vi "Measurement UI.vi"() -> ()   [LabVIEW 2025, in "Automotive Ethernet Frame Generator UI.lvlib"]
uses:
  Automotive Ethernet Frame Generator UI.lvlib
  Automotive Ethernet Frame Generator/OOB gRPC Client/OOB gRPC Client.lvlib
  <vilib>/gRPC/LabVIEW gRPC Library/Shared/grpcId.ctl
  <vilib>/gRPC/LabVIEW gRPC Library/grpc-lvsupport-release.lvlib
panel:
  out "OOB gRPC Port":i32
  out "STATUS":string
  in  "CYCLE?":bool
  in  "PAUSE PCAP PLAYBACK":bool
  in  "PCAP PLAYBACK":bool
  in  "PATH":path
  out "Protocol Layer 2":T1
  out "Payload":string
  in  "SEND FRAME":bool
  out "INTERFACE NAME":refnum<k21>
  out "SENT PACKETS":i32
  out "TC10 POWER MODE":bool
  in  "SEND TC10 COMMAND":bool
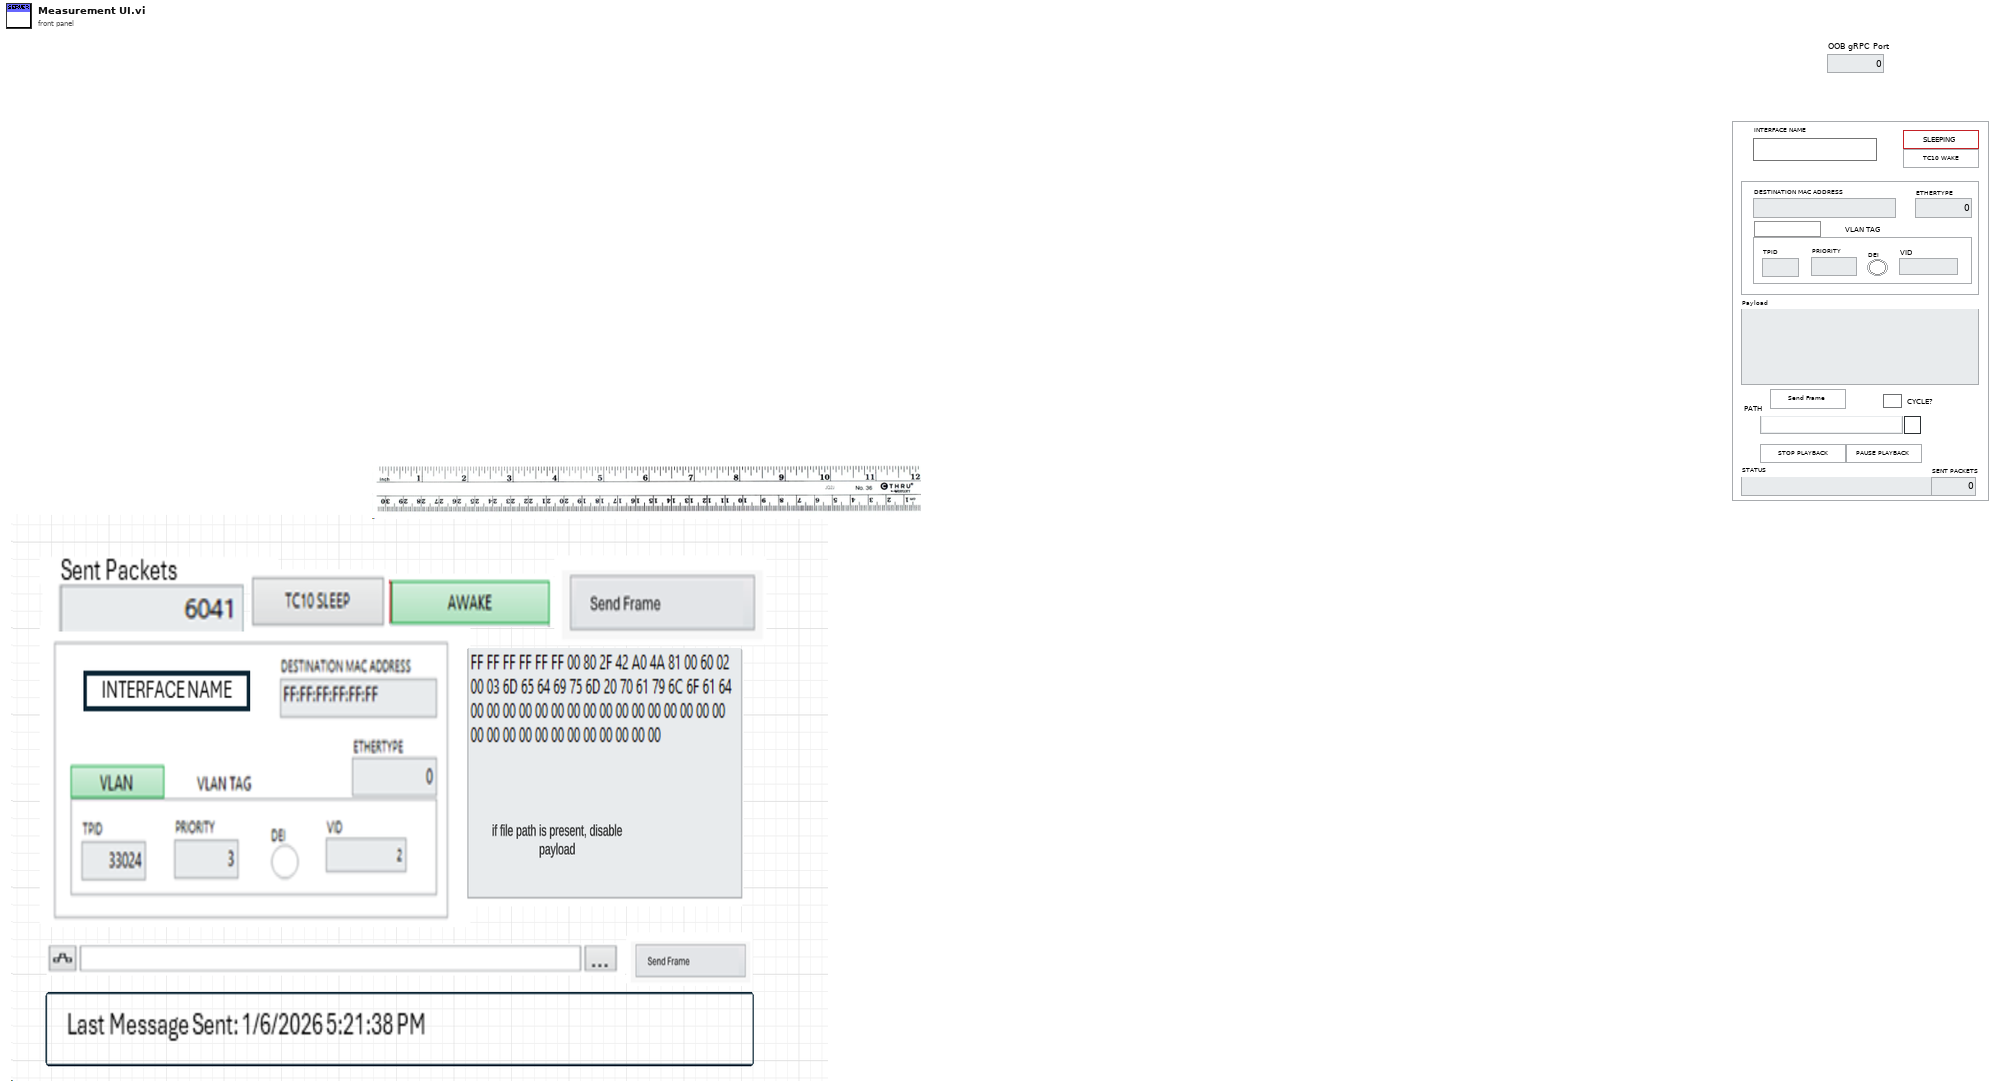
[diagram p1: front panel]
types:
  T1 = cluster{"Has VLAN":bool, "VLAN TAG":cluster{"TPID":u16, "PRIORITY":u8, "DEI":bool, "VID":u16}, "DESTINATION MAC ADDRESS":string, "ETHERTYPE":u16}
  T2 = typedef "grpc-lvsupport-release.lvlib/grpcId.ctl" = u64
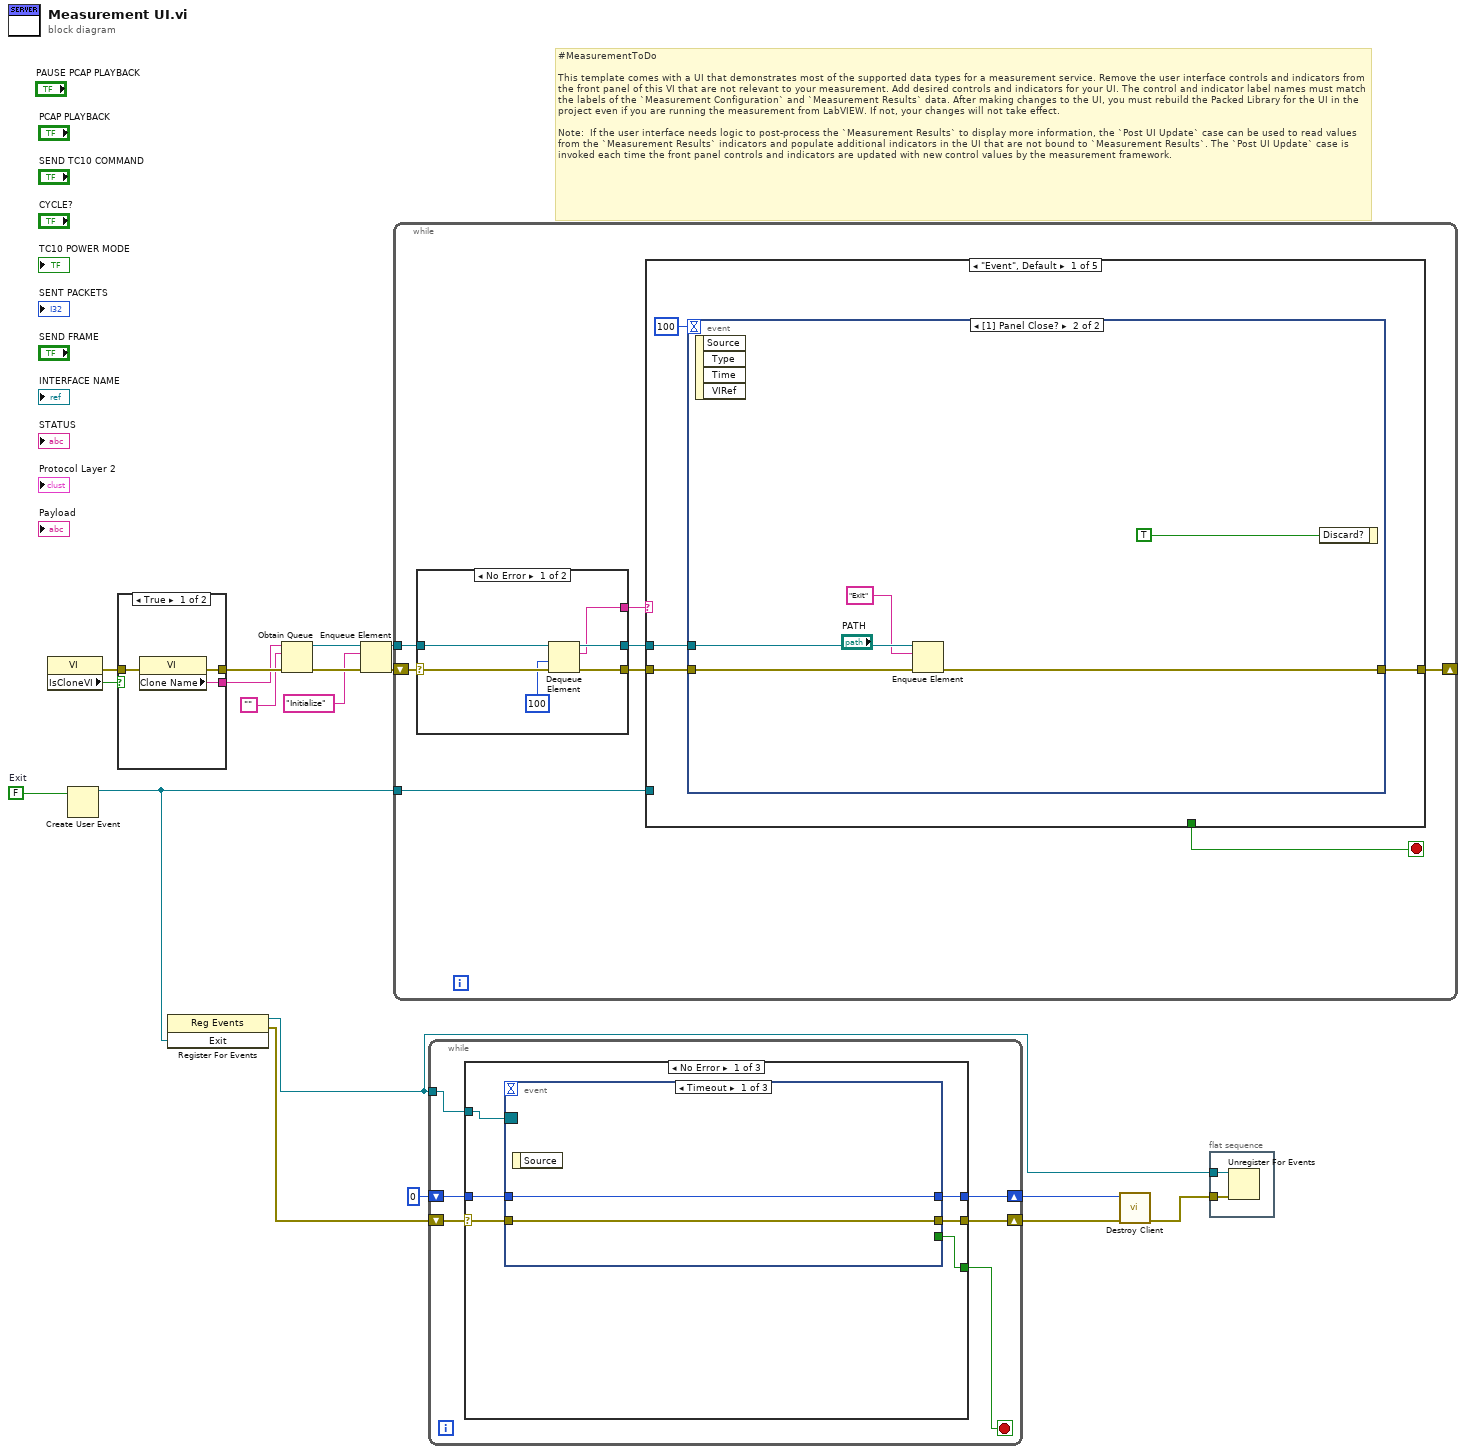
[diagram p0: block diagram]
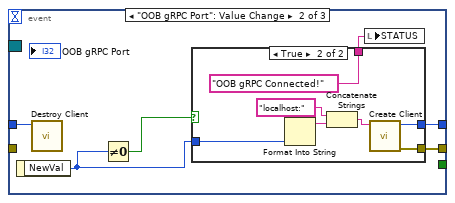
[diagram p2: hidden frame]
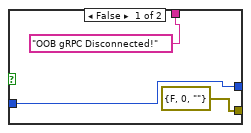
[diagram p3: hidden frame]
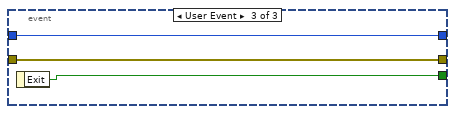
[diagram p4: hidden frame]
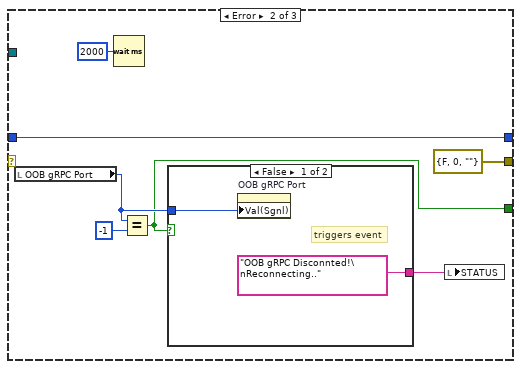
[diagram p5: hidden frame]
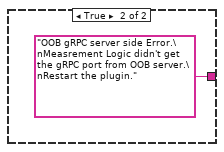
[diagram p6: hidden frame]
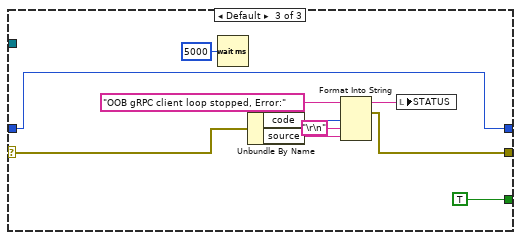
[diagram p7: hidden frame]
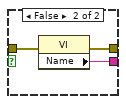
[diagram p8: hidden frame]
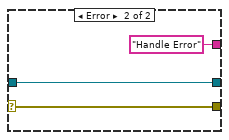
[diagram p9: hidden frame]
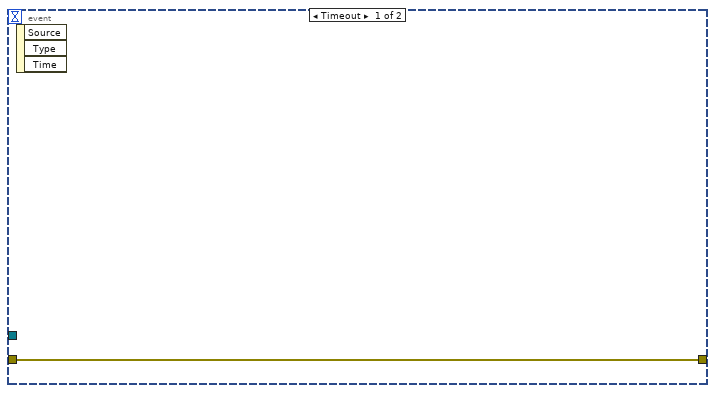
[diagram p10: hidden frame]
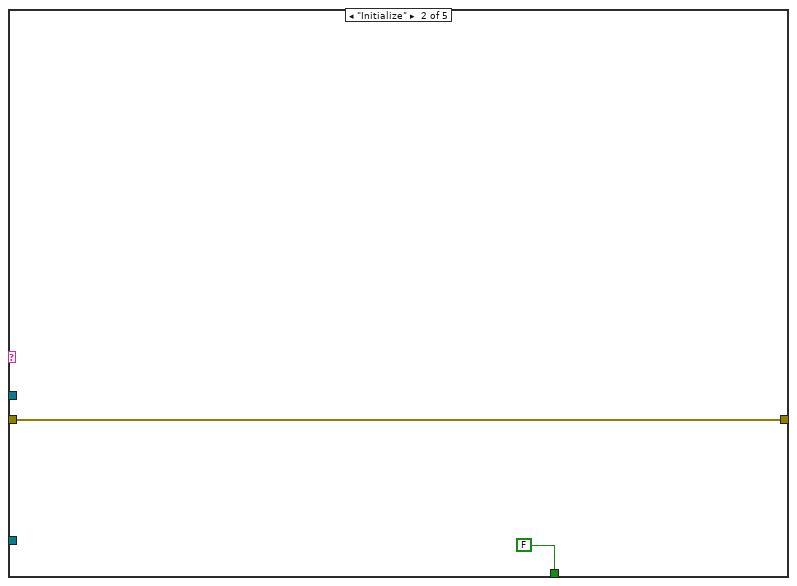
[diagram p11: hidden frame]
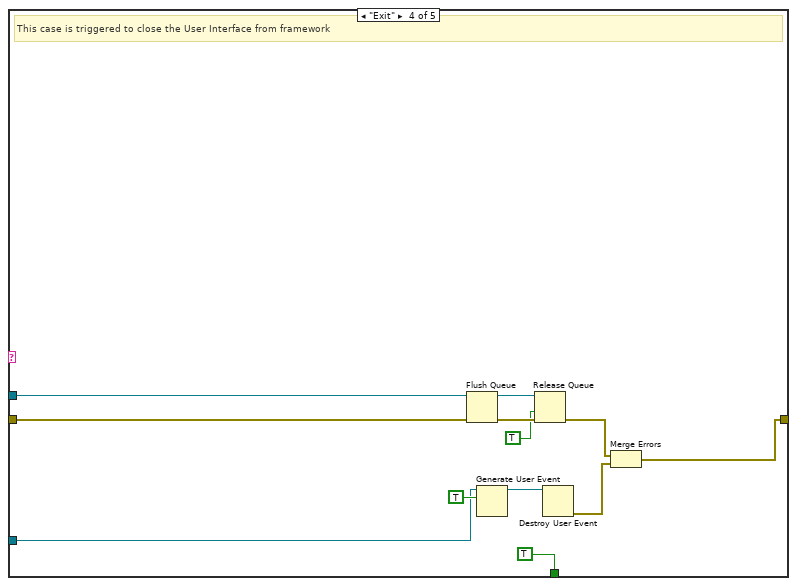
[diagram p13: hidden frame]
diagram:
  w1 = FALSE  # Exit
  # "#MeasurementToDo  \n\nThis template comes with a UI that demonstrates most of the supported data types for a measurement service. Remove the user interface controls and indicators from the front panel of this VI that are not relevant to your measurement. Add desired controls and indicators for your UI. The control and indicator label names must match the labels of the `Measurement Configuration` and `Measurement Results` data. After making changes to the UI, you must rebuild the Packed Library for the UI in the project even if you are running the measurement from LabVIEW. If not, your changes will not take effect.\n\nNote:  If the user interface needs logic to post-process the `Measurement Results` to display more information, the `Post UI Update` case can be used to read values from the `Measurement Results` indicators and populate additional indicators in the UI that are not bound to `Measurement Results`. The `Post UI Update` case is invoked each time the front panel controls and indicators are updated with new control values by the measurement framework."
  n1 = property class="VI"() -> (error out=w9:errorcluster, "IsCloneVI"=w10:bool)  [unwired: 2 in, 1 out]
  n2 = Create User Event(user event datatype=w1) -> (user event=w8:refnum<user-event>)  [unwired: 1 in, 1 out]
  n3 = case shown="True" w10 {
    tunnel: [w21 w24] -> w18
    tunnel: [w20 w23] -> w17
    tunnel: w9 -> [w19 w22]
    frame True {
      n4 = property class="VI"(error in=w19) -> (error out=w21:errorcluster, "Clone Name"=w20:string)  [unwired: 1 in, 1 out]
    }
    frame False {
      n5 = property class="VI"(error in=w22) -> (error out=w24:errorcluster, "Name"=w23:string)  [unwired: 1 in, 1 out]
    }
  }
  n6 = register-events(w8) -> (reference out=w5:refnum<event-registration>, error out=w7:errorcluster)  [unwired: 2 in]
  n7 = Obtain Queue(name (unnamed)=w17, element data type="", error in (no error)=w18) -> (queue out=w14:refnum<queue>, error out=w16:errorcluster)  [unwired: 2 in, 1 out]
  n8 = Enqueue Element(queue=w14, element="Initialize", error in (no error)=w16) -> (queue out=w13:refnum<queue>, error out=w15:errorcluster)  [unwired: 1 in, 1 out]
  n9 = while {
    shift-right: [w27] -> _
    shift-left: w15 -> [w32]
    tunnel: w13 -> [w30]
    tunnel: w8 -> [w25]
    stop <- w26 stop-if-true
    n10 = case shown="No Error" w32 {
      selector: w32 -> [w38 w41]
      tunnel: [w37 w41] -> w31
      tunnel: w30 -> [w36 w40]
      tunnel: [w35 w40] -> w29
      tunnel: [w34 "Handle Error"] -> w28
      frame No Error {
        n11 = Dequeue Element(queue=w36, timeout in ms (-1)=100, error in (no error)=w38) -> (queue out=w35:refnum<queue>, element=w34:string, error out=w37:errorcluster)  [unwired: 1 out]
      }
      frame Error {
      }
    }
    n12 = case shown="\"Event\", Default" w28 {
      tunnel: w31 -> [w44 w53 w54 w66 w67]
      tunnel: w29 -> [w42 _ _ w64 _]
      tunnel: [w45 w53 w54 w55 w67] -> w27
      tunnel: [_ FALSE _ TRUE _] -> w26
      tunnel: w25 -> [_ _ _ w56 _]
      frame "Event", Default {
        n13 = event shown="[1] Panel Close?" {
          selector: _ -> [_ _]
          dyn-events: _ -> [_ _]
          timeout: 100 -> [_ _]
          tunnel: [w46 w49] -> w45
          tunnel: w44 -> [w46 w50]
          tunnel: w42 -> [_ w48]
          event Timeout {
            n14 = event-data() -> ()  [unwired: 1 in, 3 out]
          }
          event Panel Close? {
            n15 = event-data() -> ()  [unwired: 1 in, 4 out]
            n16 = Enqueue Element(queue=w48, element="Exit", error in (no error)=w50) -> (error out=w49:errorcluster)  [unwired: 1 in, 2 out]
            n17 = event-data("Discard?"=TRUE) -> ()  [unwired: 1 in, 1 out]
          }
        }
      }
      frame "Initialize" {
      }
      frame "Post UI Update" {
        # "This case will be triggered, after framework updates the User interface with result values."
      }
      frame "Exit" {
        # "This case is triggered to close the User Interface from framework"
        n18 = Flush Queue(queue=w64, error in (no error)=w66) -> (queue out=w63:refnum<queue>, error out=w62:errorcluster)  [unwired: 1 out]
        n19 = Generate User Event(user event=w56, event data cluster=TRUE ("event data")) -> (user event out=w59:refnum<user-event>)  [unwired: 2 in, 1 out]
        n20 = Release Queue(queue=w63, force destroy? (F)=TRUE, error in (no error)=w62) -> (error out=w58:errorcluster)  [unwired: 2 out]
        n21 = Destroy User Event(user event=w59) -> (error out=w57:errorcluster)  [unwired: 1 in]
        n22 = Merge Errors(w58, w57) -> (w55:errorcluster)
      }
      frame "Handle Error" {
      }
    }
  }
  n23 = while {
    tunnel: w5 -> [w68]
    shift-right: [w72] -> w4
    shift-left: w7 -> [w73]
    shift-right: [w71] -> w3
    shift-left: T2 0 ("gRPC ID Out") -> [w70]
    stop <- w69 stop-if-true
    n24 = case shown="No Error" w73 {
      selector: w73 -> [w76 _ w114]
      tunnel: [w79 errorcluster {"status"=FALSE, "code"=0, "source"=""} ("error IO") w113] -> w72
      tunnel: [w78 w107 w115] -> w71
      tunnel: w70 -> [w77 w107 w115]
      tunnel: [w75 w101 TRUE] -> w69
      tunnel: w68 -> [w74 _ _]
      frame No Error {
        n25 = event shown="[0] Timeout" {
          selector: w74 -> [_ _ _]
          dyn-events: _ -> [_ _ _]
          timeout: _ -> [_ _ _]
          tunnel: [w80 w85 w99] -> w79
          tunnel: [w81 w84 w98] -> w78
          tunnel: w77 -> [w81 w83 w98]
          tunnel: w76 -> [w80 _ w99]
          tunnel: [_ _ w100] -> w75
          event Timeout {
            n26 = event-data() -> ()  [unwired: 1 in, 1 out]
          }
          event "OOB gRPC Port": Value Change {
            n27 = event-data() -> ("NewVal"=w86:i32)  [unwired: 1 in]
            n28 = call "Destroy Client.vi"("gRPC ID"=w83) -> ()  [unwired: 10 in, 1 out]
            n29 = Not Equal To 0?(x=w86) -> (x != 0?=w87:bool)
            n30 = case shown="True" w87 {
              tunnel: w86 -> [w88 w91]
              tunnel: [errorcluster {"status"=FALSE, "code"=0, "source"=""} ("error out") w94] -> w85
              tunnel: [w88 w93] -> w84
              tunnel: ["OOB gRPC Disconnected!" ("Status") "OOB gRPC Connected!" ("Status")] -> w82
              frame False {
              }
              frame True {
                n31 = Format Into String(w91) -> (resulting string=w97:string)  [unwired: 3 in, 1 out]
                n32 = Concatenate Strings("localhost:" ("string"), w97) -> (w95:string)
                n33 = call "Create Client.vi"("address"=w95) -> ("error out"=w94:errorcluster, "gRPC ID Out"=w93:T2)  [unwired: 9 in]
              }
            }
            n34 = local write "STATUS"(w82) -> ()
          }
          event User Event {
            n35 = event-data() -> ("Exit"=w100:bool)  [unwired: 1 in]
          }
        }
      }
      frame Error {
        n36 = local read "OOB gRPC Port"() -> (w102:i32)
        n37 = Wait (ms)(milliseconds to wait=u32 2000) -> ()  [unwired: 1 out]
        n38 = Equal?(x=w102, y=-1 ("x")) -> (x = y?=w101:bool)
        n39 = case shown="False" w101 {
          tunnel: w102 -> [w109 _]
          tunnel: ["OOB gRPC Disconnted!\nReconnecting.." ("Status") "OOB gRPC server side Error.\nMeasrement Logic didn't get the gRPC port from OOB server.\nRestart the plugin." ("Status")] -> w105
          frame False {
            # "triggers event"
            n40 = property on="OOB gRPC Port" class="DigNum (strict)"("Val(Sgnl)"=w109) -> ()  [unwired: 2 in, 2 out]
          }
          frame True {
          }
        }
        n41 = local write "STATUS"(w105) -> ()
      }
      frame Default {
        n42 = Wait (ms)(milliseconds to wait=u32 5000) -> ()  [unwired: 1 out]
        n43 = Unbundle By Name(w114) -> ("code"=w120:i32, "source"=w119:string)
        n44 = Format Into String(initial string="OOB gRPC client loop stopped, Error:" ("format string"), w120, "\r\n", w119) -> (resulting string=w111:string, error out=w113:errorcluster)  [unwired: 2 in]
        n45 = local write "STATUS"(w111) -> ()
      }
    }
  }
  n46 = call "Destroy Client.vi"("error in"=w4, "gRPC ID"=w3) -> ("error out"=w6:errorcluster)  [unwired: 9 in]
  n47 = flat-sequence {
    tunnel: w5 -> [w122]
    tunnel: w6 -> [w121]
    frame #0 {
      n48 = Unregister For Events(event registration refnum=w122, error in=w121) -> ()  [unwired: 1 out]
    }
  }
